vi "RFH-add-data_to_sim.vi"() -> ()   [LabVIEW 2020, in "RFH-Reflection_File_Handler.lvlib"]
doc: "Run by hand: adds the water or salt water model permittivity and the impedance to the simulated files of a folder and saves them. The user picks the folder and the files."
uses:
  RFH-Reflection_File_Handler.lvlib
  Computation/RDC-Reflection_Data_Computation.lvlib
panel:
  out "error out":errorcluster
  in  "Water":bool
  in  "Array 2":dbl[](array[numeric])=[10.0, 15.0, 20.0, 22.5, 25.0, 30.0, 35.0, 40.0]
  out "Array":string[](array[string])
  in  "cancel":bool
  in  "Continue":bool
  in  "folder path":path
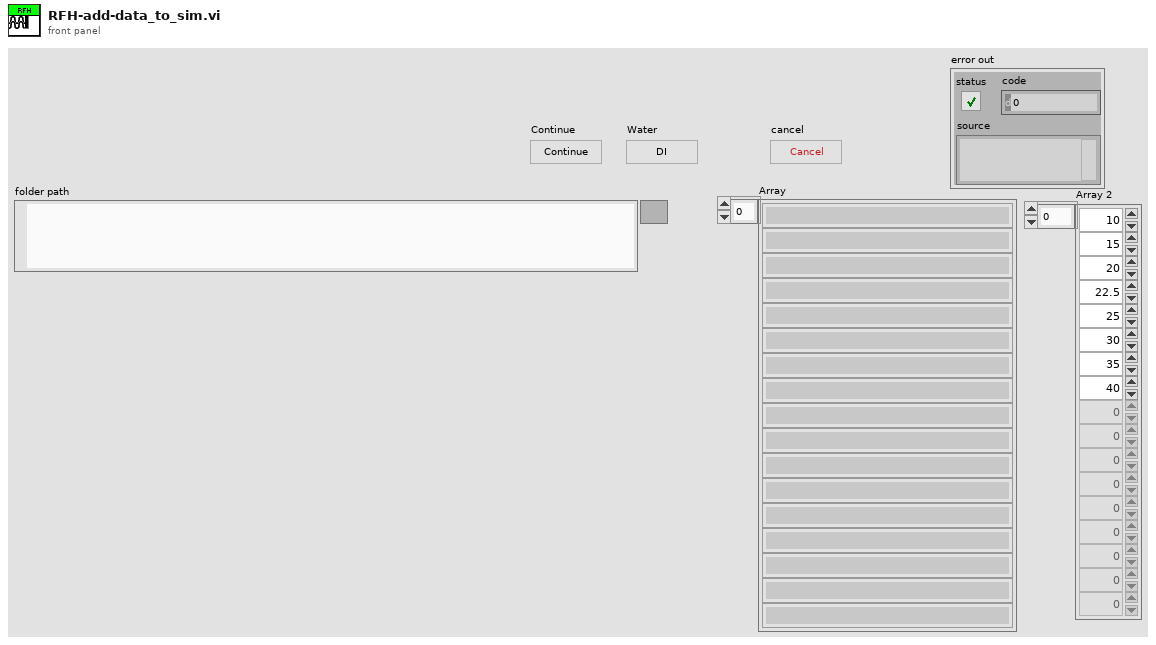
[diagram p1: front panel]
types:
  T1 = typedef "RFH-Reflection_File_Handler.lvlib/RFH-common_data_format.ctl" = cluster{"Frequency":dbl[], "Reflection'":dbl[], "Reflection''":dbl[], "Permativity'":dbl[], "Permativity''":dbl[], "Conductivity":dbl[], "Loss Tangent":dbl[], "Resistance":dbl[], "Reactance":dbl[]}
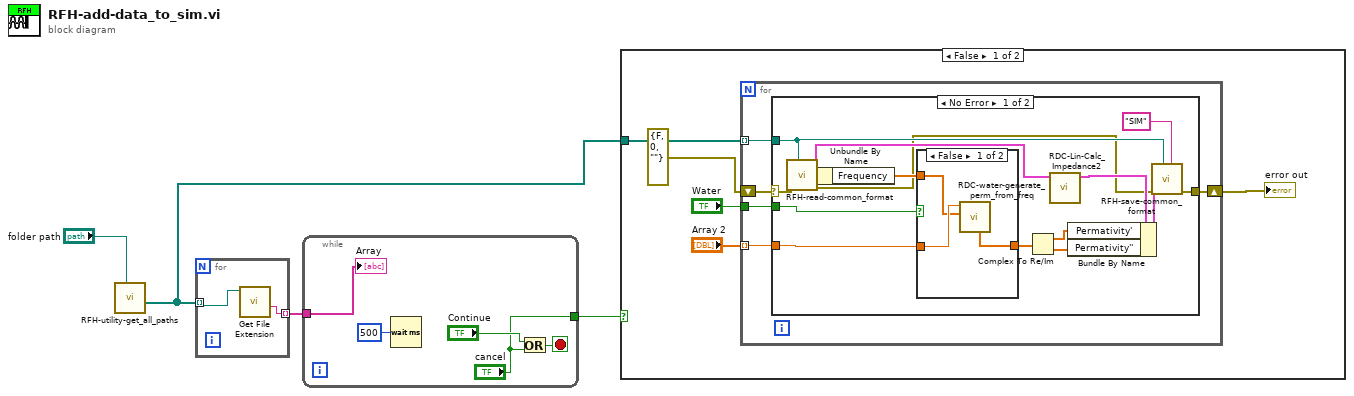
[diagram p0: block diagram]
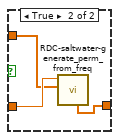
[diagram p2: hidden frame]
diagram:
  n1 = call "RFH-utility-get_all_paths.vi"("Folder Path"="folder path") -> ("All Files in Dir"=w1:path[])  [unwired: 7 in, 3 out]
  n2 = for {
    tunnel: w1 -> [w6] mode=indexing
    tunnel: [w5] -> w3 mode=indexing
    n3 = call <vilib>:"Get File Extension.vi"("file"=w6) -> ("filename without extension"=w5:string)  [unwired: 6 in, 4 out]
  }
  n4 = while {
    tunnel: ["cancel"] -> w4
    tunnel: w3 -> [w7]
    stop <- w8 stop-if-true
    n5 = Wait (ms)(milliseconds to wait=u32 500) -> ()  [unwired: 1 out]
    n6 = Or(x="Continue", y="cancel") -> (x .or. y?=w8:bool)
    "Array" <- w7
  }
  n7 = case shown="False" w4 {
    tunnel: w1 -> [w14 _]
    frame False {
      n8 = for {
        tunnel: "Water" -> [w21]
        tunnel: "Array 2" -> [w20] mode=indexing
        tunnel: w14 -> [w19] mode=indexing
        shift-right: [w18] -> w12
        shift-left: errorcluster {"status"=FALSE, "code"=0, "source"=""} ("error out") -> [w17]
        n9 = case shown="No Error" w17 {
          selector: w17 -> [w24 w42]
          tunnel: w21 -> [w35 _]
          tunnel: w20 -> [w34 _]
          tunnel: w19 -> [w32 _]
          tunnel: [w25 w42] -> w18
          frame No Error {
            n10 = call "RFH-read-common_format.vi"("file path (dialog if empty)"=w32, "error in"=w24) -> ("error out"=w23:errorcluster, "Common Format"=w31:T1)  [unwired: 8 in]
            n11 = Unbundle By Name(w31) -> ("Frequency"=w33:dbl[])
            n12 = case shown="False" w35 {
              tunnel: w34 -> [w38 w41]
              tunnel: w33 -> [w37 w40]
              tunnel: [w36 w39] -> w28
              frame False {
                n13 = call "RDC-water-generate_perm_from_freq.vi"("Frequency"=w37, "water Temp (25C) [10-40C]"=w38) -> ("Complex perm"=w36:cdb[])  [unwired: 5 in, 4 out]
              }
              frame True {
                n14 = call "RDC-saltwater-generate_perm_from_freq.vi"("Frequency"=w40, "water Temp (25C) [10-40C]"=w41) -> ("Complex perm"=w39:cdb[])  [unwired: 6 in, 3 out]
              }
            }
            n15 = Complex To Re/Im(x + iy=w28) -> (x=w27:dbl[], y=w26:dbl[])
            n16 = call "RDC-Lin-Calc_Impedance2.vi"("input cluster"=w31) -> ("Output cluster"=w30:T1)  [unwired: 9 in, 1 out]
            n17 = Bundle By Name(cluster=w30, "Permativity'"=w27, "Permativity''"=w26) -> (w29:T1)
            n18 = call "RFH-save-common_format.vi"("source"="SIM", "file path (use dialog)"=w32, "error in (no error)"=w23, "Common Format"=w29) -> ("error out"=w25:errorcluster)  [unwired: 7 in]
          }
          frame Error {
          }
        }
      }
      "error out" <- w12
    }
    frame True {
    }
  }
